vi "CE Center - Error Handler.vi"(6 "error before":errorcluster, 8 "CE message":string, 9 "CE error status":bool) -> (0 "error out":errorcluster)   [LabVIEW 2021]
doc: "::: CalcExpress Toolkit :::\nCopyright (c) 2000-2026 Konstantin Shifershteyn. All rights reserved."
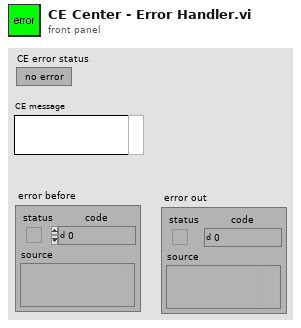
[diagram p1: front panel]
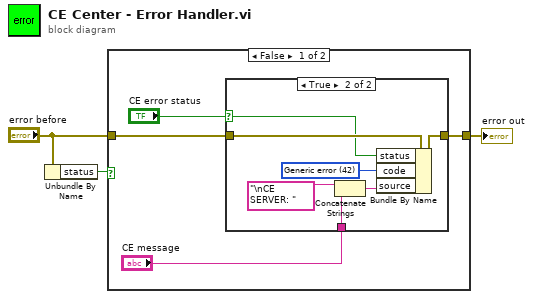
[diagram p0: block diagram]
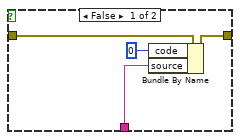
[diagram p2: hidden frame]
diagram:
  n1 = Unbundle By Name("error before") -> ("status"=w2:bool)
  n2 = case shown="False" w2 {
    tunnel: "error before" -> [w7 w19]
    tunnel: [w6 w19] -> w3
    frame False {
      n3 = case shown="True" "CE error status" {
        selector: "CE error status" -> [_ w12]
        tunnel: w7 -> [w11 w18]
        tunnel: [w10 w17] -> w6
        tunnel: "CE message" -> [w8 w13]
        frame False {
          n4 = Bundle By Name(cluster=w11, "code"=0, "source"=w8) -> (w10:errorcluster)
        }
        frame True {
          w14 = u16 42 items=["No error", "Argument error", "Memory is full", "Out of zone", "End of file", "File already open", "Generic file I/O error", "File not found", "File permission error", "Disk is full", "Duplicate path", "Too many files open", "System feature not enabled", "Resource file not found", "Cannot add resource", "Resource not found", "Image not found", "Image memory error", "Pen does not exist", "Config type invalid", "Config token not found", "Config parse error", "Config memory error", "Bad external code format", "Bad external code offset", "External code not present", "Null window", "Destroy window error", "Null menu", "Print aborted", "Bad print record", "Print driver error", "Windows error during printing", "Memory error during printing", "Print dialog error", "Generic print error", "Invalid device refnum", "Device not found", "Device parameter error", "Device unit error", "Cannot open device", "Device call aborted", "Generic error", "Cancelled by user", "Object ID too low", "Object ID too high", "Object not in heap", "Unknown heap", "Unknown object (invalid DefProc)", "Unknown object (DefProc not in table)", "Message out of range", "Invalid (null) method", "Unknown message", "Manager call not supported", "Bad address", "Network operation in progress", "Network operation timed out", "Connection is busy", "Network attribute not supported", "Network error", "Address in use", "System out of memory", "Connection aborted", "Connection refused", "Not connected", "Already connected", "Connection closed", "Initialization error (interapplication manager)", "Bad occurrence", "Wait on unbound occurrence handler", "Occurrence queue overflow", "Datalog type conflict", "Unused", "Unrecognized type (interapplication manager)", "Memory corrupt", "Failed to make temporary DLL", "Old CIN version", "Drag socket not found", "Failed to load drop-object", "Failed to register OLE object", "Failed to release OLE object", "Format specifier type mismatch", "Unknown format specifier", "Too few format specifiers", "Too many format specifiers", "Scan failed", "Newer CIN version", "OLE Convert", "Runtime menu error", "Password tampered", "Unknown error code"]
          n5 = Concatenate Strings("\nCE SERVER: " ("source"), w13) -> (w15:string)
          n6 = Bundle By Name(cluster=w18, "status"=w12, "code"=w14, "source"=w15) -> (w17:errorcluster)
        }
      }
    }
    frame True {
    }
  }
  "error out" <- w3
